vi "MSG display box two buttons.vi"(8 "error in":errorcluster, 9 "Enable":bool=TRUE, 10 "input string":string) -> (0 "error out":errorcluster, 1 "OK Button 2":bool, 3 "Panel close":bool)   [LabVIEW 2021]
panel:
  in  "Text.Text Colors:BG Color":u32(colorbox)=16448250
  out "String Indicator":string
  in  "OK Button":bool
  in  "Cancel":bool
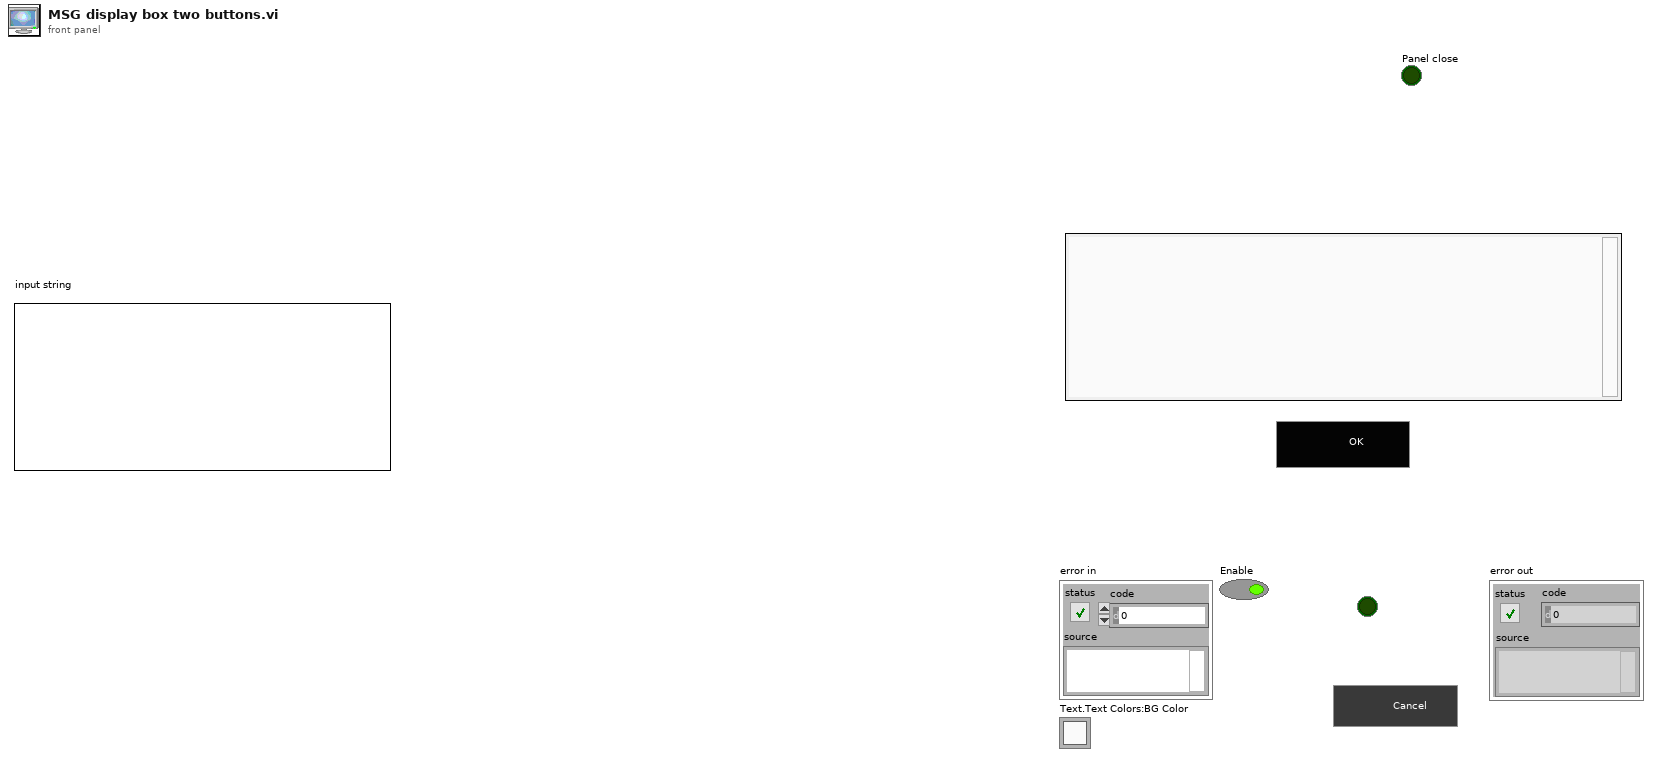
[diagram p1: front panel]
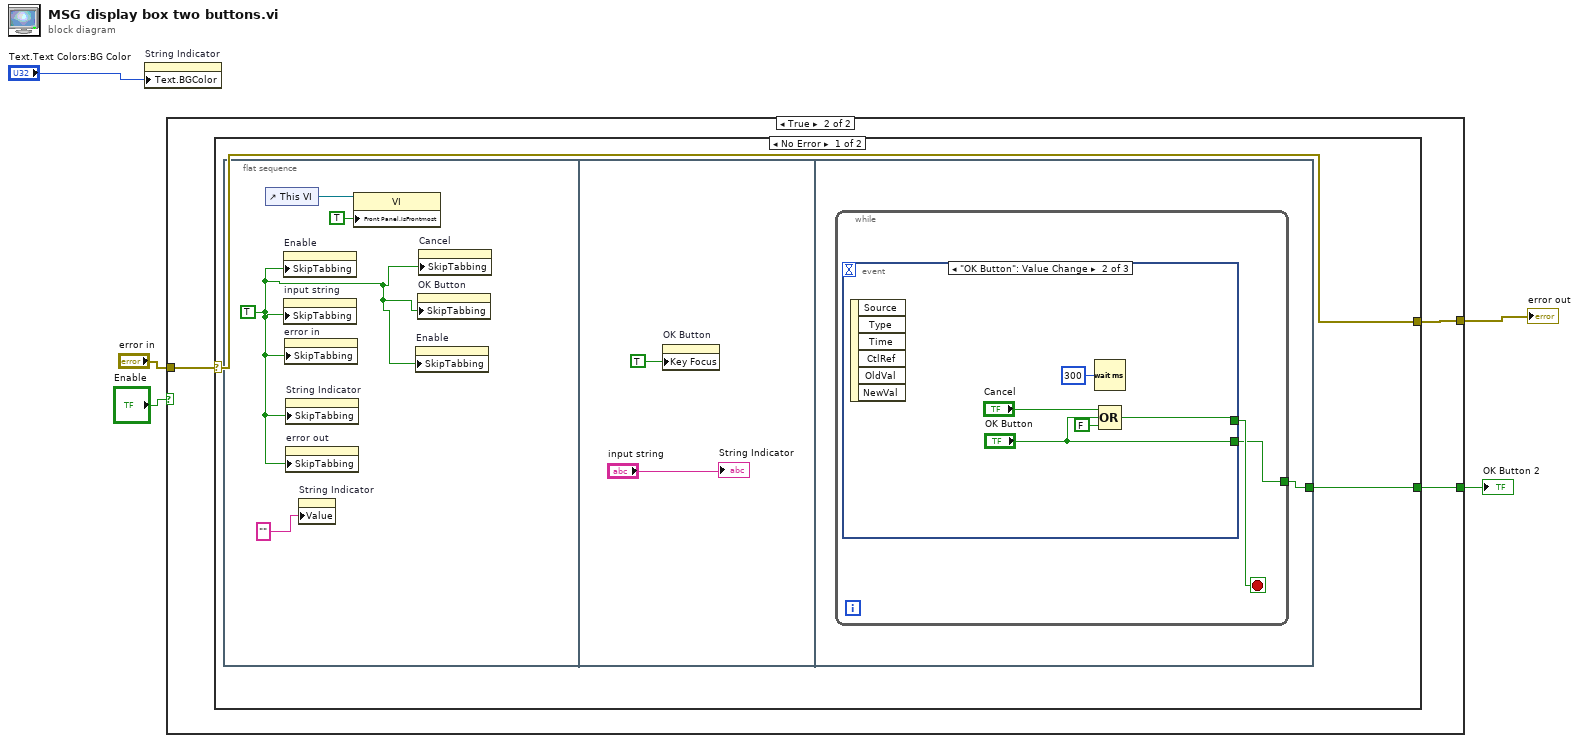
[diagram p0: block diagram]
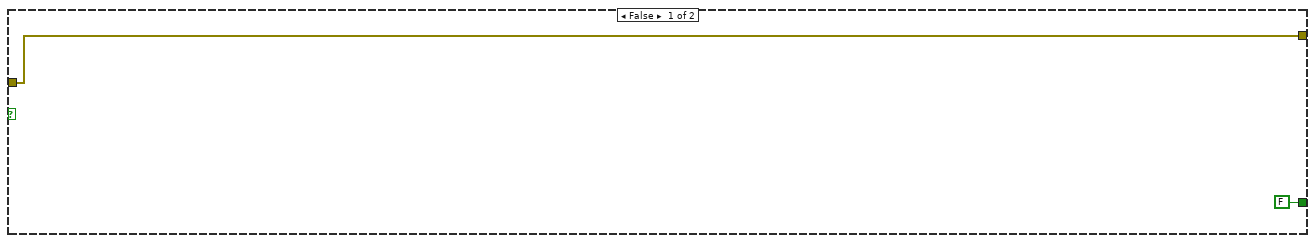
[diagram p2: hidden frame]
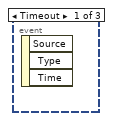
[diagram p3: hidden frame]
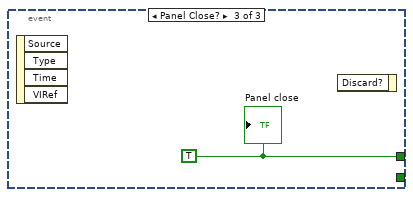
[diagram p4: hidden frame]
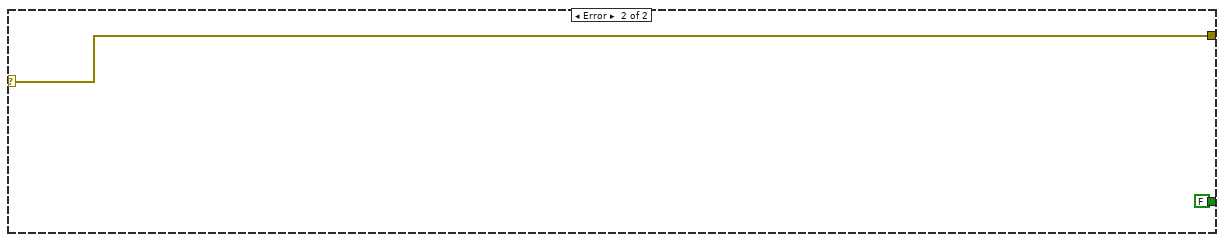
[diagram p5: hidden frame]
diagram:
  n1 = property on="String Indicator" class="Str"("Text.BGColor"="Text.Text Colors:BG Color") -> ()  [unwired: 2 in, 2 out]
  n2 = case shown="True" "Enable" {
    tunnel: "error in" -> [w7 w10]
    tunnel: [w7 w9] -> w4
    tunnel: [FALSE ("OK Button") w8] -> w1
    frame False {
    }
    frame True {
      n3 = case shown="No Error" w10 {
        selector: w10 -> [w12 w29]
        tunnel: [w12 w29] -> w9
        tunnel: [w11 FALSE ("OK Button")] -> w8
        frame No Error {
          n4 = flat-sequence {
            tunnel: [w19] -> w11
            frame #0 {
              w14 = TRUE ("Skip When Tabbing")
              n5 = control-ref of="This VI"() -> (w16:refnum<vi>)
              n6 = property on="Enable" class="Bool (strict)"("SkipTabbing"=w14) -> ()  [unwired: 2 in, 2 out]
              n7 = property on="input string" class="Str"("SkipTabbing"=w14) -> ()  [unwired: 2 in, 2 out]
              n8 = property on="error in" class="Clust (strict)"("SkipTabbing"=w14) -> ()  [unwired: 2 in, 2 out]
              n9 = property on="String Indicator" class="Str"("SkipTabbing"=w14) -> ()  [unwired: 2 in, 2 out]
              n10 = property on="error out" class="Clust (strict)"("SkipTabbing"=w14) -> ()  [unwired: 2 in, 2 out]
              n11 = property on="String Indicator" class="Str"("Value"="" ("String Indicator")) -> ()  [unwired: 2 in, 2 out]
              n12 = property class="VI"(reference=w16, "Front Panel.IsFrontmost"=TRUE ("Front Panel Window:Is Frontmost")) -> ()  [unwired: 1 in, 2 out]
              n13 = property on="Enable" class="Bool (strict)"("SkipTabbing"=w14) -> ()  [unwired: 2 in, 2 out]
              n14 = property on="OK Button" class="Bool"("SkipTabbing"=w14) -> ()  [unwired: 2 in, 2 out]
              n15 = property on="Cancel" class="Bool"("SkipTabbing"=w14) -> ()  [unwired: 2 in, 2 out]
            }
            frame #1 {
              n16 = property on="OK Button" class="Bool"("Key Focus"=TRUE) -> ()  [unwired: 2 in, 2 out]
              "String Indicator" <- "input string"
            }
            frame #2 {
              n17 = while {
                tunnel: [w20] -> w19
                stop <- w21 stop-if-true
                n18 = event shown="[1] \"OK Button\": Value Change" {
                  selector: _ -> [_ _ _]
                  dyn-events: _ -> [_ _ _]
                  timeout: _ -> [_ _ _]
                  tunnel: [_ w23 w27] -> w21
                  tunnel: [_ "OK Button" _] -> w20
                  event Timeout {
                    n19 = event-data() -> ()  [unwired: 1 in, 3 out]
                  }
                  event "OK Button": Value Change {
                    n20 = event-data() -> ()  [unwired: 1 in, 6 out]
                    n21 = Wait (ms)(milliseconds to wait=u32 300) -> ()  [unwired: 1 out]
                    n22 = Compound Arithmetic op=OR("Cancel", "OK Button", FALSE ("value")) -> (w23:bool)
                  }
                  event Panel Close? {
                    w27 = TRUE
                    n23 = event-data() -> ()  [unwired: 1 in, 4 out]
                    n24 = event-data() -> ()  [unwired: 2 in, 1 out]
                    "Panel close" <- w27
                  }
                }
              }
            }
          }
        }
        frame Error {
        }
      }
    }
  }
  "error out" <- w4
  "OK Button 2" <- w1
